vi "rt-test.vi"() -> ()   [LabVIEW 2020]
uses:
  <vilib>/xnet/xnet.llb/XNET Convert.vi
  <vilib>/xnet/xnet.llb/XNET Convert (Signal to Frame CAN).vi
  Addon Engine/SubVI/CAN Frames Write.vi
  Addon Engine/SubVI/CAN Frames Read.vi
  <vilib>/xnet/xnet.llb/XNET Convert (Frame CAN to Signal).vi
  <vilib>/FPGAPlugInAG/Dynamic/niLvFpga_Close_Dynamic.vi
  <vilib>/rvi/interface/nirviCloseFPGA/nirviCloseFPGA.xnode
  Addon Engine/Types/FPGA Refnum.ctl
  Addon Engine/985x Support Addon Engine.lvlib
  <vilib>/rvi/interface/nirviReadWriteControl/nirviReadWriteControl.xnode
  <vilib>/rvi/interface/Simulation/niFpgaSimulationCallBeginRW.vi
  <vilib>/rvi/errors/niLvFpgaAdjustHostInterfaceError.vi
panel:
  out "CAN1_Tx":u32[](array[numeric]) format="%.0x"
  out "CAN1_Rx":u32[](array[numeric]) format="%.0x"
  out "CAN0_Tx":u32[](array[numeric]) format="%.0x"
  out "CAN0_Rx":u32[](array[numeric]) format="%.0x"
  in  "CAN0":dbl[](array[numeric])=[1.0, 2.0] caption="signal data" format="%.2f"
  in  "Write":bool
  out "error out":errorcluster
  in  "stop":bool
  out "CAN1":dbl[](array[numeric]) caption="signal data" format="%.2f"
  in  "signal list":refnum<k21>[](array[refnum])=["CANEventSignal1\nNIXNET_example.CAN_Cluster", "CANCyclicSignal2\nnixnet_example.CAN_Cluster"]
  in  "Bitfile path":path=path "c:/ni-rt/VeriStand/Custom Devices/FPGA Addon/985xsupport_FPGATarget_fpga-main_5XgmTEdlmQU.lvbitx"
  in  "Device address":string="RIO0"
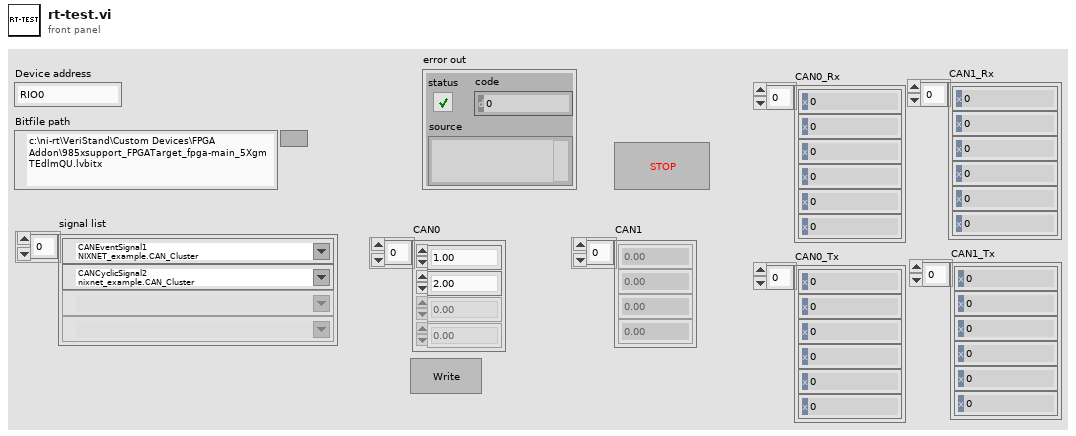
[diagram p1: front panel]
types:
  T1 = typedef "985x Support Addon Engine.lvlib/FPGA Refnum.ctl" = refnum<k20>
  T2 = typedef "985x Support Addon Engine.lvlib/Tx Event Session.ctl" = cluster{"FPGA Refnum":T1, "Channel Number":u32, "Conv Session":refnum<k21>}
  T3 = typedef "985x Support Addon Engine.lvlib/Rx Session.ctl" = cluster{"FPGA Refnum":T1, "Channel Number":u32, "Conv Session":refnum<k21>, "Signal ID":u32[], "Signals DVR":refnum<data-value>}
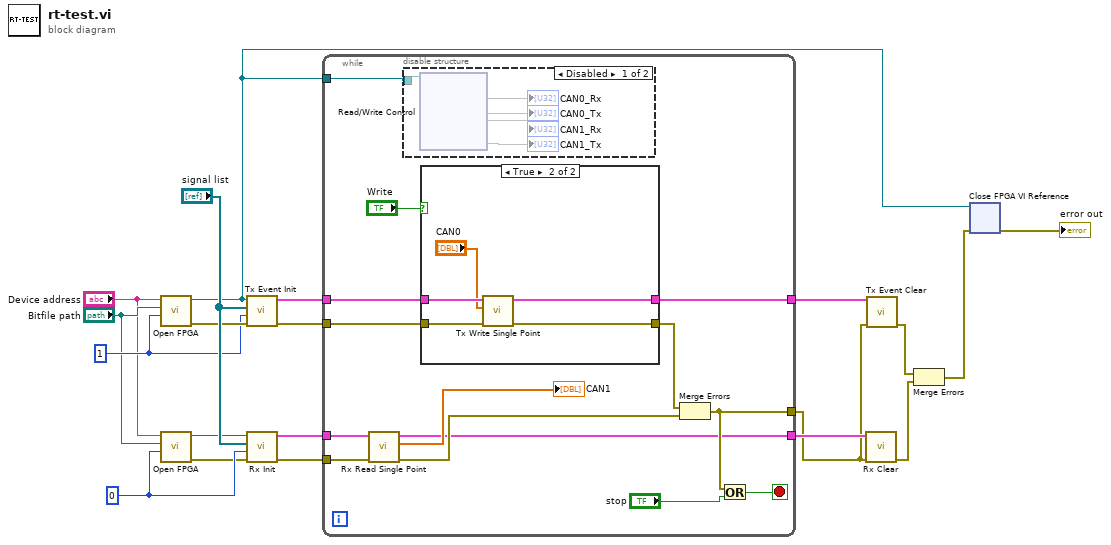
[diagram p0: block diagram]
diagram:
  w6 = u32 1 ("Channel Number")
  w3 = u32 0 ("Channel Number")
  n1 = call "Open FPGA.vi"("Channel Number"=w6, "Bitfile path"="Bitfile path", "Device address"="Device address") -> ("error out"=w8:errorcluster, "Bitfile reference out"=w2:T1)  [unwired: 7 in]
  n2 = call "Open FPGA.vi"("Channel Number"=w3, "Bitfile path"="Bitfile path", "Device address"="Device address") -> ("error out"=w1:errorcluster, "Bitfile reference out"=w7:T1)  [unwired: 7 in]
  n3 = call "Tx Event Init.vi"("error in (no error)"=w8, "Channel Number"=w6, "signal list"="signal list", "FPGA Refnum"=w2) -> ("error out"=w15:errorcluster, "Tx Event"=w16:T2)  [unwired: 6 in]
  n4 = call "Rx Init.vi"("error in (no error)"=w1, "Channel Number"=w3, "signal list"="signal list", "FPGA Refnum"=w7) -> ("error out"=w19:errorcluster, "Rx Session"=w17:T3)  [unwired: 6 in]
  n5 = while {
    tunnel: [w32] -> w13
    tunnel: w19 -> [w31]
    tunnel: w17 -> [w27]
    tunnel: [w28] -> w18
    tunnel: w16 -> [w25]
    tunnel: w15 -> [w24]
    tunnel: [w23] -> w14
    tunnel: w2 -> [w21]
    stop <- w34 stop-if-true
    n6 = call "Rx Read Single Point.vi"("error in (no error)"=w31, "Rx Session In"=w27) -> ("error out"=w29:errorcluster, "Data"=→"CAN1":dbl[], "Rx Session Out"=w28:T3)  [unwired: 7 in]
    n7 = disable-structure shown="Disabled" {
      disable-tunnel: w21 -> [w39 _]
      frame Disabled {
        n8 = xnode "Read/Write Control"("FPGA VI Reference In"=w39) -> ("CAN0_Rx"=→"CAN0_Rx", "CAN0_Tx"=→"CAN0_Tx", "CAN1_Rx"=→"CAN1_Rx", "CAN1_Tx"=→"CAN1_Tx")  [unwired: 1 in, 2 out]
      }
      frame Enabled {
      }
    }
    n9 = case shown="True" "Write" {
      tunnel: w25 -> [w41 w46]
      tunnel: w24 -> [w40 w44]
      tunnel: [w41 w43] -> w23
      tunnel: [w40 w42] -> w22
      frame False {
      }
      frame True {
        n10 = call "Tx Write Single Point.vi"("error in (no error)"=w44, "Outgoing data"="CAN0", "Tx Event In"=w46) -> ("error out"=w42:errorcluster, "Tx Event Out"=w43:T2)  [unwired: 7 in]
      }
    }
    n11 = Merge Errors(w22, w29) -> (w32:errorcluster)
    n12 = Or(x=w32, y="stop") -> (x .or. y?=w34:bool)
  }
  n13 = call "Rx Clear.vi"("error in (no error)"=w13, "Rx Session In"=w18) -> ("error out"=w11:errorcluster)  [unwired: 9 in]
  n14 = call "Tx Event Clear.vi"("error in (no error)"=w13, "Tx Event"=w14) -> ("error out"=w12:errorcluster)  [unwired: 9 in]
  n15 = Merge Errors(w12, w11) -> (w10:errorcluster)
  n16 = xnode "Close FPGA VI Reference"("FPGA VI Reference In"=w2, "error in"=w10) -> ("error out"=→"error out":errorcluster)
